vi "Create Panel by Type.vi"(5 "Display Type":refnum<class "ArrayPanel.lvclass">, 7 "Panel Type":refnum<class "ArrayPanel.lvclass">, 8 "error in (no error)":errorcluster, 9 "Run? (T)":bool=TRUE, 11 "PanelArray in":refnum<class "ArrayManager.lvclass">) -> (0 "error out":errorcluster, 2 "Panel":refnum<class "ArrayPanel.lvclass">, 3 "PanelArray out":refnum<class "ArrayManager.lvclass">)   [LabVIEW 2020, in "OOPanel.lvlib" / "ArrayManager.lvclass"]
uses:
  ArrayManager.lvclass
  ArrayPanel/ArrayPanel.lvclass
  C:/dev/LabVIEW/lv-oopanel/OOPanel/Panel/Panel.lvclass
  ArrayManager.lvclass/ArrayManager.ctl
  ArrayPanel/ArrayPanel.lvclass/ArrayPanel.ctl
  Manager/Manager.lvclass
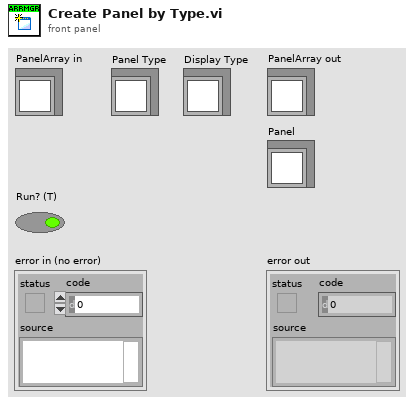
[diagram p1: front panel]
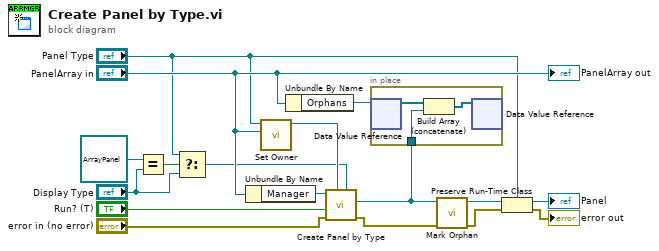
[diagram p0: block diagram]
diagram:
  n1 = Equal?(x=refnum<class "ArrayPanel.lvclass"> refnum, y="Display Type") -> (x = y?=w4:bool)
  n2 = Select(t="Panel Type", s=w4, f="Display Type") -> (s? t:f=w1:refnum<class "ArrayPanel.lvclass">)
  n3 = Unbundle By Name("PanelArray in") -> ("Manager"=w17:refnum<class "Manager.lvclass">)
  n4 = call "Set Owner.vi"("Owner"="PanelArray in", "ArrayPanel in"="Panel Type") -> ("ArrayPanel out"=w9:refnum<class "ArrayPanel.lvclass">)  [unwired: 8 in, 1 out]
  n5 = Unbundle By Name("PanelArray in") -> ("Orphans"=w12:refnum<data-value>)
  n6 = call "Create Panel by Type.vi"("Display Class Type"=w1, "Panel Type"=w9, "error in (no error)"="error in (no error)", "Run? (T)"="Run? (T)", "Manager in"=w17) -> ("error out"=w6:errorcluster, "Panel"=w7:refnum<class "ArrayPanel.lvclass">)  [unwired: 4 in, 1 out]
  n7 = in-place {
    in-place-border: w7 -> [w19]
    n8 = in-place-dvr #1(w12) -> (w20:refnum<class "ArrayPanel.lvclass">[])  [unwired: 1 out]
    n9 = Build Array (concatenate)(w20, w19) -> (w18:refnum<class "ArrayPanel.lvclass">[])
    n10 = in-place-dvr #1(w18) -> ()  [unwired: 2 out]
  }
  n11 = call "Mark Orphan.vi"("error in (no error)"=w6, "ArrayPanel in"=w7) -> ("error out"=w10:errorcluster, "ArrayPanel out"=w11:refnum<class "ArrayPanel.lvclass">)  [unwired: 8 in]
  n12 = Preserve Run-Time Class(object in=w11, error in=w10, 2:"Panel Type") -> (object out=→"Panel":refnum<class "ArrayPanel.lvclass">, error out=→"error out":errorcluster)
  "PanelArray out" <- "PanelArray in"
